vi "Main.vi"(11 "Module Admin":refnum<class "Delacor_lib_QMH_Module Admin.lvclass">) -> ()   [LabVIEW 2018, in "Log_class.lvlib"]
doc: "This template is based off of the Queued Message Handler design pattern and the Queued Message Handler project template that ships with LabVIEW.\n\nThe main difference is that the queue is private to this module and communication between modules is performed via Broadcast and Request events.\n\nRequest events are wrapped in public API methods and are handled in the Event Handling Loop (EHL) of this VI. Any module can register for Broadcast events sent by this module. The EHL generates messages based on user interface actions.\n\nThe Message Handling Loop (MHL) processes messages generated by the EHL, or by other messages. The messages are string values, so new messages can be added easily to the Message Cases case structure in the MHL. Each message cluster can also provide an optional value for Message Data, which is a variant that can be converted to whatever message-specific data is required.\n_____\nBased on DQMH Dev Tools: Project Template 7.1.1.1528."
uses:
  Log_class.lvlib
  <vilib>/Delacor/Delacor QMH/Libraries/Module Admin_class/Delacor_lib_QMH_Module Admin.lvclass
  Register_logs.ctl
  Module Data--cluster.ctl
  <vilib>/Delacor/Delacor QMH/Libraries/Message Queue_class/Delacor_lib_QMH_Message Queue.lvclass/Delacor_lib_QMH_Message Queue.ctl
  Stop Argument--cluster.ctl
  <vilib>/Delacor/Delacor QMH/Libraries/Module Admin_class/Delacor_lib_QMH_Module Admin.lvclass/Delacor_lib_QMH_Module Admin.ctl
  Log recording Argument--cluster.ctl
  Storage method changed Argument--cluster.ctl
  Request logs Argument--cluster.ctl
  Request logs (Reply Payload)--cluster.ctl
  Request save Argument--cluster.ctl
  <vilib>/Utility/miscctls.llb/LVPointTypeDef.ctl
  <vilib>/Delacor/Delacor QMH/Libraries/Message Queue_class/Delacor_lib_QMH_Enqueue Message (Single).vi
  <vilib>/Delacor/Delacor QMH/Libraries/Module Admin_class/Delacor_lib_QMH_Get External Launch.vi
  <vilib>/Delacor/Delacor QMH/Libraries/Message Queue_class/Delacor_lib_QMH_Message Queue.lvclass
panel:
  out "枚举":enum16{"自动存储", "触发式存储"}(ring)
  in  "组合框":T1
  out "error out":errorcluster
  out "Status":string
  in  "Simulate MHL Error":bool
  in  "Simulate EHL Error":bool
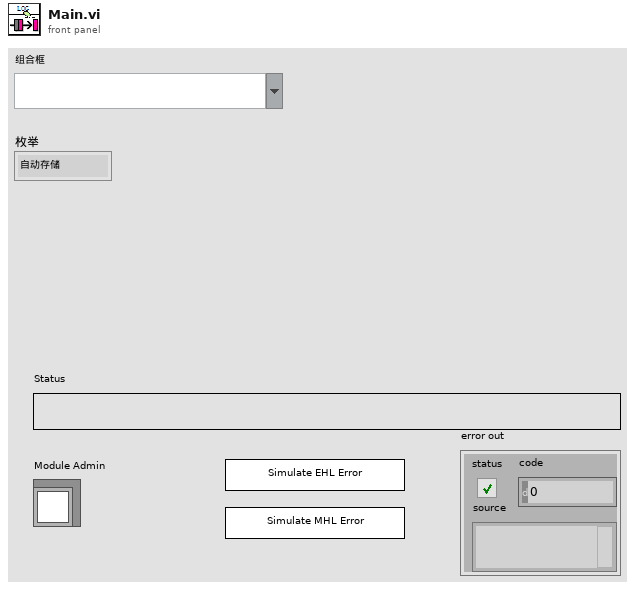
[diagram p1: front panel]
types:
  T1 = typedef "Log_class.lvlib/Register_logs.ctl" = string
  T2 = typedef "Log_class.lvlib/Request Events--cluster.ctl" = cluster{"Stop Module":refnum<user-event>, "Show Panel":refnum<user-event>, "Hide Panel":refnum<user-event>, "Get Module Execution Status":refnum<user-event>, "Show Diagram":refnum<user-event>, "记录日志":refnum<user-event>, "存储方式更改":refnum<user-event>, "请求日志":refnum<user-event>, "请求保存":refnum<user-event>}
  T3 = typedef "Log_class.lvlib/Module Data--cluster.ctl" = cluster{"Status":string, "创建的日志名":string[], "日志内容":string[], "存储方式":enum16{"自动存储", "触发式存储"}}
  T4 = enum32{"invalid lock state", "Not Locked", "Locked (No Password)", "Password-protected"}
  T5 = typedef "Log_class.lvlib/Stop Argument--cluster.ctl" = cluster{"Origin":string, "Exit via Stop Module Req?":bool, "Wait for Module to stop?":bool}
  T6 = typedef "Log_class.lvlib/Log recording Argument--cluster.ctl" = cluster{"日志选择":T1, "日志内容":string}
  T7 = typedef "Log_class.lvlib/Storage method changed Argument--cluster.ctl" = cluster{"枚举":enum16{"自动存储", "触发式存储"}}
  T8 = typedef "Log_class.lvlib/Request logs Argument--cluster.ctl" = cluster{"组合框":T1, "Wait Notifier":refnum<notifier>, "wait for reply":bool}
  T9 = typedef "Log_class.lvlib/Request save Argument--cluster.ctl" = cluster{"要保存的日志":T1}
  T10 = typedef "LVPointTypeDef.ctl" = cluster{"Horizontal":i16, "Vertical":i16}
  T11 = enum32{"Invalid", "Standard", "Closed", "Hidden", "Minimized", "Maximized"}
  T12 = typedef "Log_class.lvlib/Request logs (Reply Payload)--cluster.ctl" = cluster{"日志内容":string, "error":errorcluster}
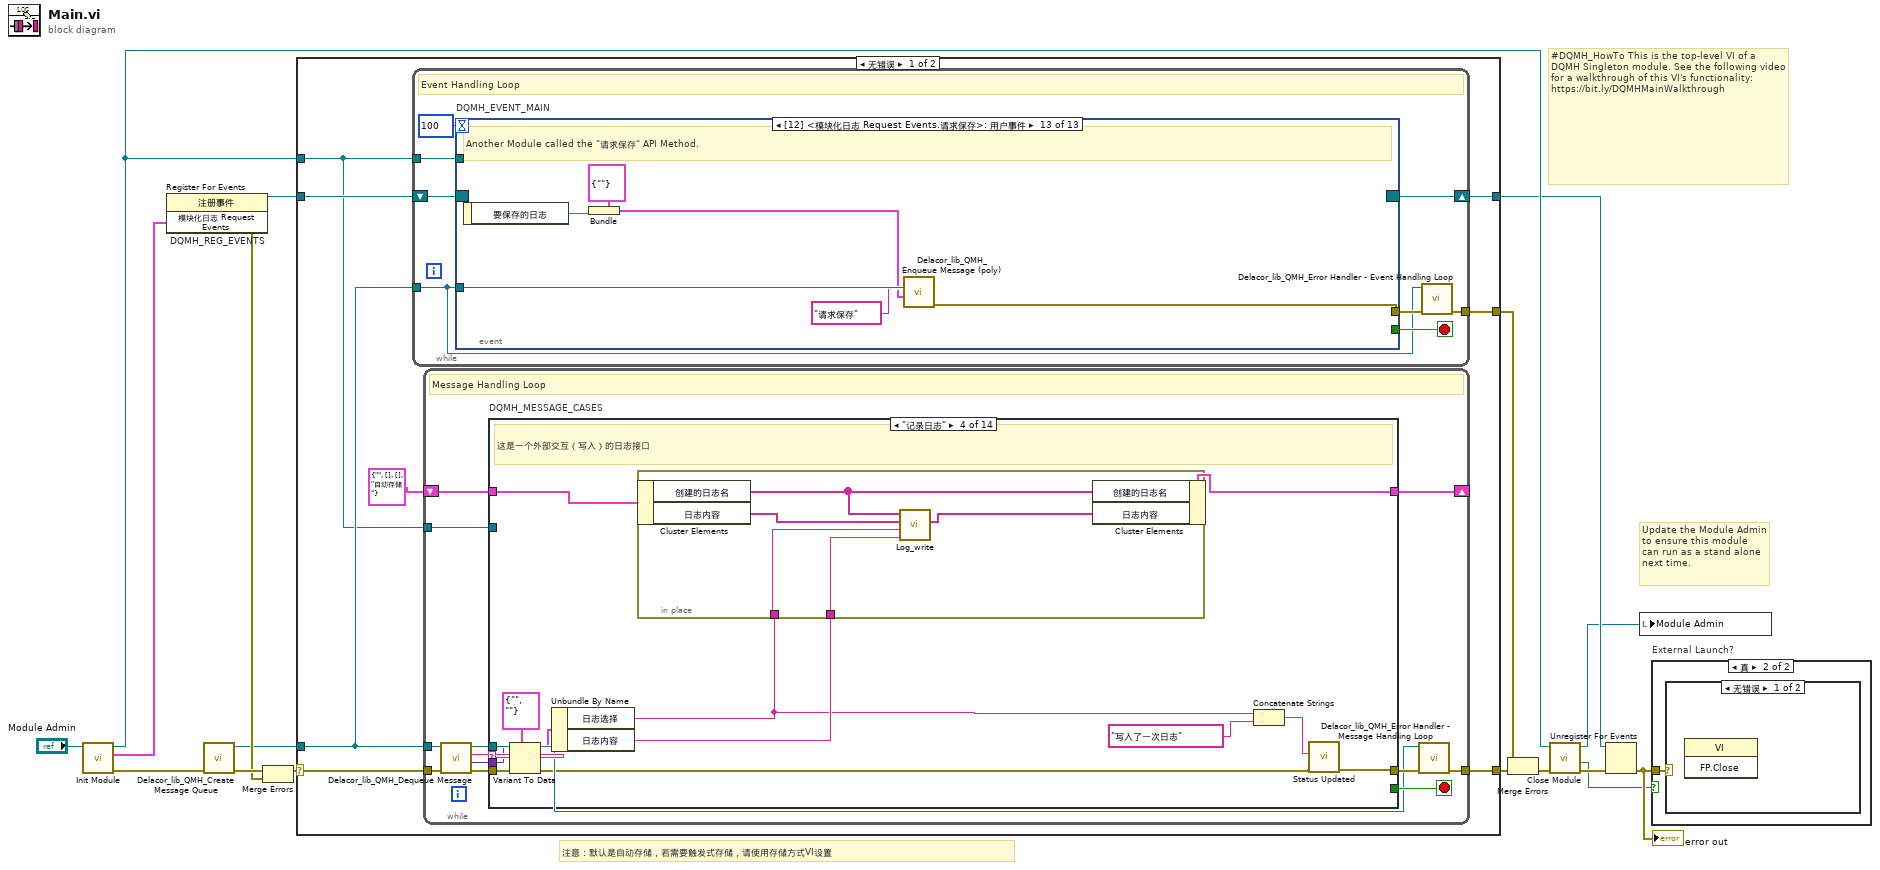
[diagram p0: block diagram]
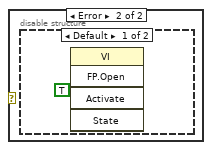
[diagram p3: hidden frame]
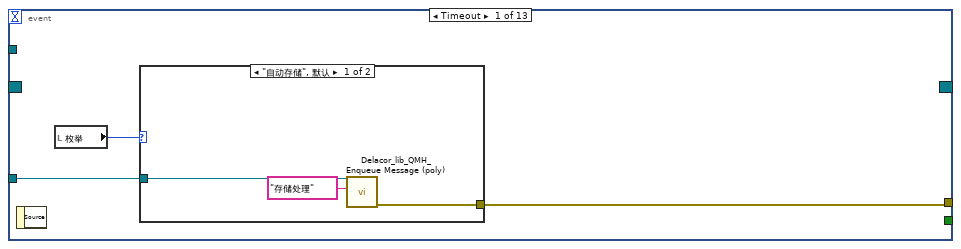
[diagram p5: hidden frame]
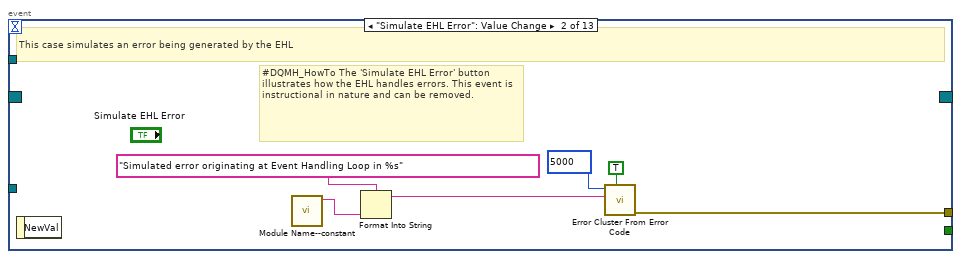
[diagram p7: hidden frame]
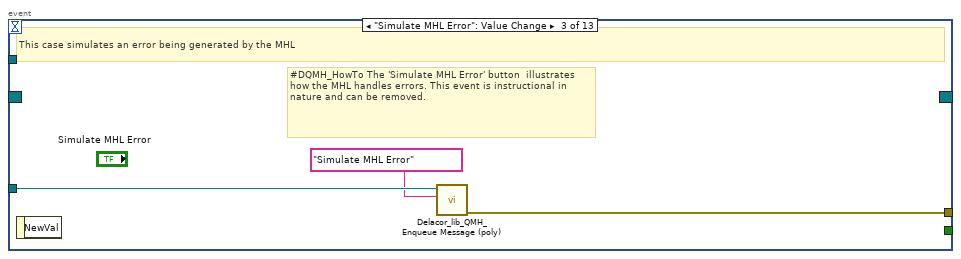
[diagram p8: hidden frame]
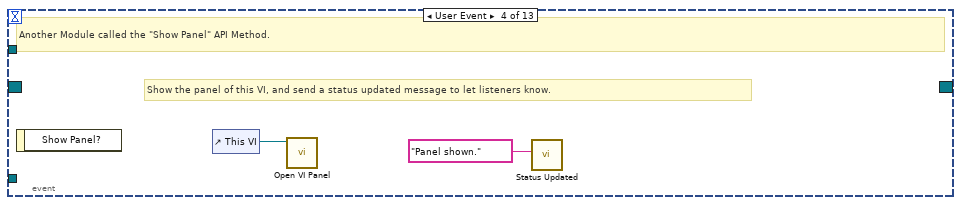
[diagram p9: hidden frame]
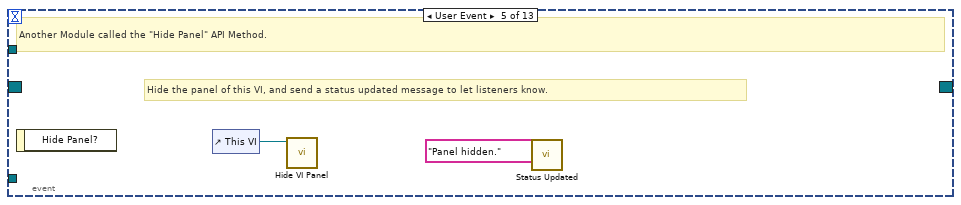
[diagram p10: hidden frame]
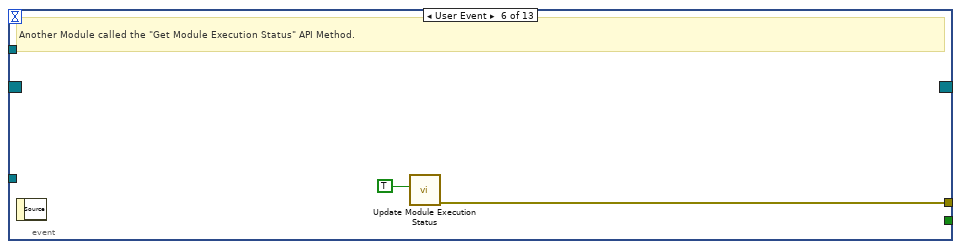
[diagram p11: hidden frame]
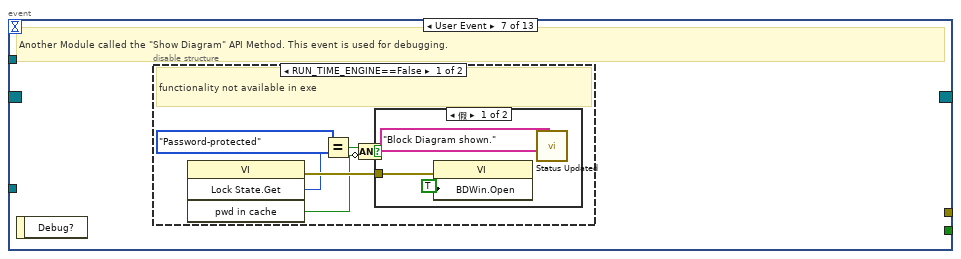
[diagram p12: hidden frame]
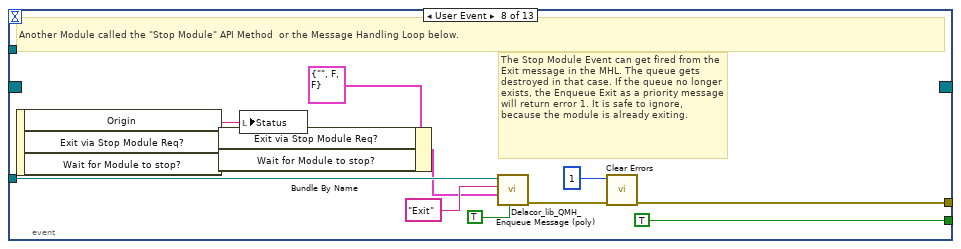
[diagram p15: hidden frame]
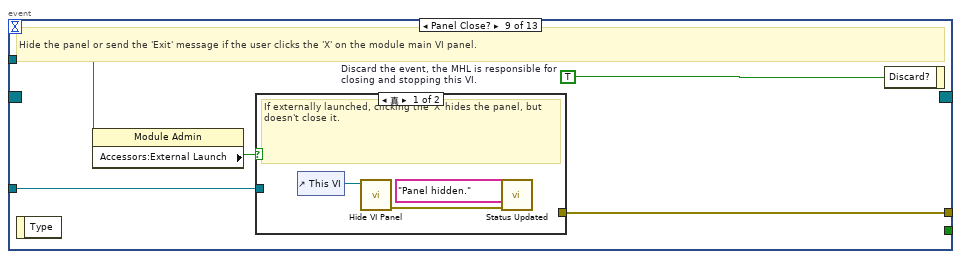
[diagram p16: hidden frame]
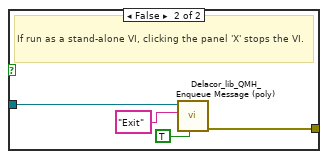
[diagram p17: hidden frame]
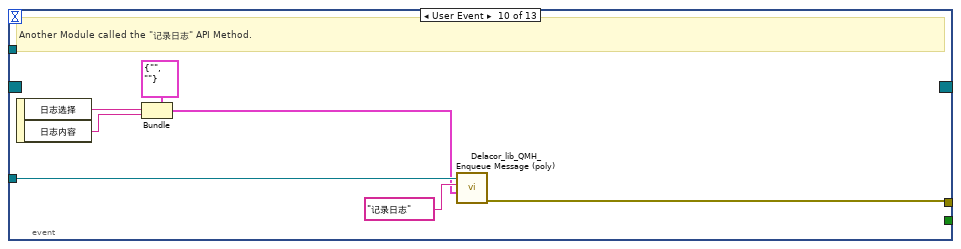
[diagram p18: hidden frame]
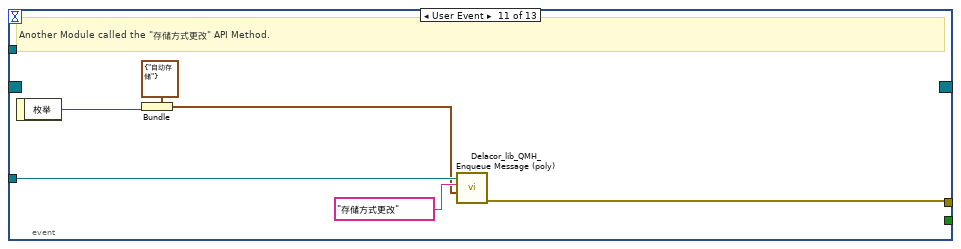
[diagram p19: hidden frame]
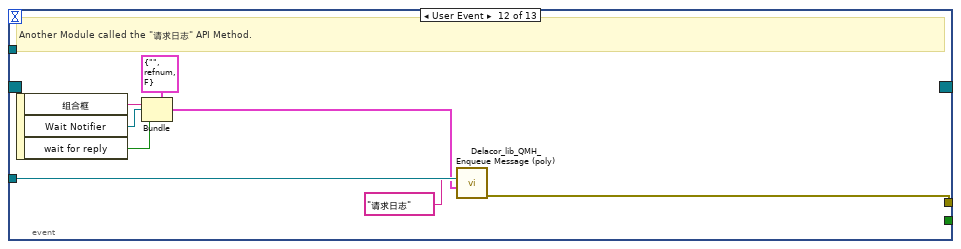
[diagram p20: hidden frame]
diagram:
  # "注意：默认是自动存储，若需要触发式存储，请使用存储方式VI设置"
  # "#DQMH_HowTo This is the top-level VI of a DQMH Singleton module. See the following video for a walkthrough of this VI's functionality: https://bit.ly/DQMHMainWalkthrough"
  # "Update the Module Admin to ensure this module can run as a stand alone next time."
  n1 = call "Init Module.vi"("Singleton Module Admin in"="Module Admin") -> ("error out"=w16:errorcluster, "模块化日志 Request Events"=w5:T2, "Singleton Module Admin out"=w8:refnum<class "Delacor_lib_QMH_Module Admin.lvclass">)  [unwired: 8 in]
  n2 = register-events "DQMH_REG_EVENTS"(w5) -> (reference out=w6:refnum<event-registration>, error out=w9:errorcluster)  [unwired: 2 in]
  n3 = call <vilib>:"Delacor_lib_QMH_Create Message Queue.vi"("error in"=w16) -> ("error out"=w11:errorcluster, "Message Queue"=w4:refnum<class "Delacor_lib_QMH_Message Queue.lvclass">)  [unwired: 9 in]
  n4 = Merge Errors(w11, w9) -> (w10:errorcluster)
  n5 = case shown="无错误" w10 {
    selector: w10 -> [w23 w297]
    tunnel: [w25 w296] -> w17
    tunnel: [w22 w295] -> w7
    tunnel: w6 -> [w20 w295]
    tunnel: w4 -> [w19 w290]
    tunnel: [w24 _] -> w14
    tunnel: w8 -> [w18 w291]
    frame No Error {
      n6 = while {
        tunnel: w19 -> [w27]
        shift-right: [w30] -> w22
        shift-left: w20 -> [w31]
        tunnel: [w32] -> w24
        tunnel: w18 -> [w28]
        stop <- w29 stop-if-true
        # "Event Handling Loop"
        n7 = event "DQMH_EVENT_MAIN" shown="[12] <模块化日志 Request Events.请求保存>: 用户事件" {
          selector: w31 -> [_ _ _ _ _ _ _ _ _ _ _ _ _]
          dyn-events: [_ _ _ _ _ _ _ _ _ _ _ _ _] -> w30
          timeout: 100 -> [_ _ _ _ _ _ _ _ _ _ _ _ _]
          tunnel: [_ _ _ _ _ _ _ TRUE ("Discard?") _ _ _ _ _] -> w29
          tunnel: w27 -> [w35 _ w47 _ _ _ _ w71 w78 w94 w100 w108 w114]
          tunnel: [w34 w45 w48 _ _ w54 _ w74 w80 w88 w95 w101 w109] -> w33
          tunnel: w28 -> [_ _ _ _ _ _ _ _ w77 _ _ _ _]
          event Timeout {
            n8 = event-data() -> ()  [unwired: 1 in, 1 out]
            n9 = local read "枚举"() -> (w36:enum16{"自动存储", "触发式存储"})
            n10 = case "条件结构" shown="\"自动存储\", 默认" w36 {
              tunnel: w35 -> [w39 _]
              tunnel: [w38 _] -> w34
              frame "自动存储", Default {
                n11 = call-poly <vilib>:"Delacor_lib_QMH_Enqueue Message (poly).vi"("Message"="存储处理", "Message Queue in"=w39) -> ("error out"=w38:errorcluster)  [unwired: 8 in, 1 out]
              }
              frame "触发式存储" {
              }
            }
          }
          event "Simulate EHL Error": Value Change {
            # "#DQMH_HowTo The 'Simulate EHL Error' button  illustrates how the EHL handles errors. This event is instructional in nature and can be removed."
            # "This case simulates an error being generated by the EHL"
            n12 = event-data() -> ()  [unwired: 1 in, 1 out]
            n13 = call "Module Name--constant.vi"() -> ("Module Name"=w42:string)  [unwired: 11 in]
            n14 = Format Into String(format string="Simulated error originating at Event Handling Loop in %s", w42) -> (resulting string=w43:string)  [unwired: 2 in, 1 out]
            n15 = call <vilib>:"Error Cluster From Error Code.vi"("show call chain? (False)"=TRUE, "error message (\"\")"=w43, "error code (0)"=5000) -> ("error out"=w45:errorcluster)  [unwired: 6 in]
          }
          event "Simulate MHL Error": Value Change {
            # "#DQMH_HowTo The 'Simulate MHL Error' button  illustrates how the MHL handles errors. This event is instructional in nature and can be removed."
            # "This case simulates an error being generated by the MHL"
            n16 = event-data() -> ()  [unwired: 1 in, 1 out]
            n17 = call-poly <vilib>:"Delacor_lib_QMH_Enqueue Message (poly).vi"("Message"="Simulate MHL Error", "Message Queue in"=w47) -> ("error out"=w48:errorcluster)  [unwired: 8 in, 1 out]
          }
          event User Event {
            # "Show the panel of this VI, and send a status updated message to let listeners know."
            # "Another Module called the \"Show Panel\" API Method."
            n18 = event-data() -> ()  [unwired: 1 in, 1 out]
            n19 = control-ref of="This VI"() -> (w50:refnum<vi>)
            n20 = call "Open VI Panel.vi"("VI"=w50) -> ()  [unwired: 10 in, 1 out]
            n21 = call "Status Updated.vi"("Status"="Panel shown." ("format string")) -> ()  [unwired: 10 in, 1 out]
          }
          event User Event {
            # "Hide the panel of this VI, and send a status updated message to let listeners know."
            # "Another Module called the \"Hide Panel\" API Method."
            n22 = event-data() -> ()  [unwired: 1 in, 1 out]
            n23 = control-ref of="This VI"() -> (w52:refnum<vi>)
            n24 = call "Hide VI Panel.vi"("VI"=w52) -> ()  [unwired: 10 in, 1 out]
            n25 = call "Status Updated.vi"("Status"="Panel hidden." ("format string")) -> ()  [unwired: 10 in, 1 out]
          }
          event User Event {
            # "Another Module called the \"Get Module Execution Status\" API Method."
            n26 = event-data() -> ()  [unwired: 1 in, 1 out]
            n27 = call "Update Module Execution Status.vi"("Running?"=TRUE) -> ("error out"=w54:errorcluster)  [unwired: 10 in]
          }
          event User Event {
            # "Another Module called the \"Show Diagram\" API Method. This event is used for debugging."
            n28 = event-data() -> ()  [unwired: 1 in, 1 out]
            n29 = disable-structure shown="RUN_TIME_ENGINE==False" {
              frame condition #0 (active) {
                # "functionality not available in exe"
                n30 = invoke on="Invoke Node" class="VI" method="Lock State.Get"() -> (error out=w60:errorcluster, "Get Lock State"=w59:T4, "pwd in cache"=w56:bool)  [unwired: 4 in, 1 out]
                n31 = Equal?(x=T4."Password-protected", y=w59) -> (x = y?=w57:bool)
                n32 = Compound Arithmetic op=AND(w57, invert w56) -> (w55:bool)
                n33 = case shown="假" w55 {
                  tunnel: w60 -> [w63 _]
                  frame False {
                    n34 = property on="Property Node" class="VI"(error in=w63, "BDWin.Open"=TRUE ("Block Diagram Window:Open")) -> ()  [unwired: 1 in, 2 out]
                    n35 = call "Status Updated.vi"("Status"="Block Diagram shown." ("format string")) -> ()  [unwired: 10 in, 1 out]
                  }
                  frame True {
                    # "Password-protected VI, and the password is not in the cache. Do not show the diagram."
                  }
                }
              }
              frame condition #1 {
              }
            }
          }
          event User Event {
            # "The Stop Module Event can get fired from the Exit message in the MHL. The queue gets destroyed in that case. If the queue no longer exists, the Enqueue Exit as a priority message will return error 1. It is safe to ignore, because the module is already exiting."
            # "Another Module called the \"Stop Module\" API Method  or the Message Handling Loop below."
            n36 = event-data() -> ("Origin"=w70:string, "Exit via Stop Module Req?"=w66:bool, "Wait for Module to stop?"=w65:bool)  [unwired: 1 in]
            n37 = Bundle By Name(cluster=T5 {"Origin"="", "Exit via Stop Module Req?"=FALSE, "Wait for Module to stop?"=FALSE} ("Stop Argument"), "Exit via Stop Module Req?"=w66, "Wait for Module to stop?"=w65) -> (w64:T5)
            n38 = local write "Status"(w70) -> ()
            n39 = call-poly <vilib>:"Delacor_lib_QMH_Enqueue Message (poly).vi"("Priority Message? (F)"=TRUE, "Message Data"=w64, "Message"="Exit", "Message Queue in"=w71) -> ("error out"=w75:errorcluster)  [unwired: 6 in, 1 out]
            n40 = call <vilib>:"Clear Errors.vi"("error in (no error)"=w75, "specific error code to clear (0: all)"=1) -> ("error out"=w74:errorcluster)  [unwired: 4 in, 1 out]
          }
          event Panel Close? {
            w79 = TRUE  # Discard the event, the MHL is responsible for closing and stopping this VI.
            # "Hide the panel or send the 'Exit' message if the user clicks the 'X' on the module main VI panel."
            n41 = event-data() -> ()  [unwired: 1 in, 1 out]
            n42 = property on="Property Node" class="Module Admin"(reference=w77) -> ("Accessors:External Launch"=w76:bool)  [unwired: 1 in, 2 out]
            n43 = case shown="真" w76 {
              tunnel: w78 -> [_ w86]
              tunnel: [_ w87] -> w80
              frame True {
                # "If externally launched, clicking the 'X' hides the panel, but doesn't close it."
                n44 = control-ref of="This VI"() -> (w83:refnum<vi>)
                n45 = call "Hide VI Panel.vi"("VI"=w83) -> ("error out"=w81:errorcluster)  [unwired: 10 in]
                n46 = call "Status Updated.vi"("error in"=w81, "Status"="Panel hidden." ("format string")) -> ()  [unwired: 9 in, 1 out]
              }
              frame False {
                # "If run as a stand-alone VI, clicking the panel 'X' stops the VI."
                n47 = call-poly <vilib>:"Delacor_lib_QMH_Enqueue Message (poly).vi"("Priority Message? (F)"=TRUE, "Message"="Exit", "Message Queue in"=w86) -> ("error out"=w87:errorcluster)  [unwired: 7 in, 1 out]
              }
            }
            n48 = event-data ("Event Filter Node")("Discard?"=w79) -> ()  [unwired: 1 in, 1 out]
          }
          event User Event {
            # "Another Module called the \"记录日志\" API Method."
            n49 = event-data() -> ("日志选择"=w90:T1, "日志内容"=w89:string)  [unwired: 1 in]
            n50 = Bundle(cluster=T6 {"日志选择"="", "日志内容"=""} ("记录日志 Argument"), "日志选择"=w90, "日志内容"=w89) -> (w91:T6)
            n51 = call-poly <vilib>:"Delacor_lib_QMH_Enqueue Message (poly).vi"("Message Data"=w91, "Message"="记录日志", "Message Queue in"=w94) -> ("error out"=w88:errorcluster)  [unwired: 7 in, 1 out]
          }
          event User Event {
            # "Another Module called the \"存储方式更改\" API Method."
            n52 = event-data() -> ("枚举"=w96:enum16{"自动存储", "触发式存储"})  [unwired: 1 in]
            n53 = Bundle(cluster=T7 {"枚举"=enum."自动存储"} ("存储方式更改 Argument"), "枚举"=w96) -> (w97:T7)
            n54 = call-poly <vilib>:"Delacor_lib_QMH_Enqueue Message (poly).vi"("Message Data"=w97, "Message"="存储方式更改", "Message Queue in"=w100) -> ("error out"=w95:errorcluster)  [unwired: 7 in, 1 out]
          }
          event User Event {
            # "Another Module called the \"请求日志\" API Method."
            n55 = event-data() -> ("组合框"=w104:T1, "Wait Notifier"=w103:refnum<notifier>, "wait for reply"=w102:bool)  [unwired: 1 in]
            n56 = Bundle(cluster=T8 {"组合框"="", "Wait Notifier"=refnum, "wait for reply"=FALSE} ("请求日志 Argument"), "组合框"=w104, "Wait Notifier"=w103, "wait for reply"=w102) -> (w105:T8)
            n57 = call-poly <vilib>:"Delacor_lib_QMH_Enqueue Message (poly).vi"("Message Data"=w105, "Message"="请求日志", "Message Queue in"=w108) -> ("error out"=w101:errorcluster)  [unwired: 7 in, 1 out]
          }
          event User Event {
            # "Another Module called the \"请求保存\" API Method."
            n58 = event-data() -> ("要保存的日志"=w110:T1)  [unwired: 1 in]
            n59 = Bundle(cluster=T9 {"要保存的日志"=""} ("请求保存 Argument"), "要保存的日志"=w110) -> (w111:T9)
            n60 = call-poly <vilib>:"Delacor_lib_QMH_Enqueue Message (poly).vi"("Message Data"=w111, "Message"="请求保存", "Message Queue in"=w114) -> ("error out"=w109:errorcluster)  [unwired: 7 in, 1 out]
          }
        }
        n61 = call-dynamic "Delacor_lib_QMH_Error Handler - Event Handling Loop.vi"("error in"=w33, "Message Queue in"=w27) -> ("dup error in"=w32:errorcluster)  [unwired: 8 in, 1 out]
      }
      n62 = while {
        tunnel: w19 -> [w115]
        shift-right: [w123] -> _
        shift-left: T3 {"Status"="", "创建的日志名"=[], "日志内容"=[], "存储方式"=enum."自动存储"} ("Data Cluster") -> [w124]
        tunnel: w23 -> [w126]
        tunnel: [w118] -> w25
        tunnel: w18 -> [w119]
        stop <- w122 stop-if-true
        # "Message Handling Loop"
        n63 = call-dynamic "Delacor_lib_QMH_Dequeue Message.vi"("error in"=w126, "Message Queue in"=w115) -> ("error out"=w125:errorcluster, "Message Data"=w120:variant, "Message"=w121:string, "Message Queue out"=w116:refnum<class "Delacor_lib_QMH_Message Queue.lvclass">)  [unwired: 6 in]
        n64 = case "DQMH_MESSAGE_CASES" shown="\"记录日志\"" w121 {
          selector: w121 -> [_ _ _ _ _ _ _ _ _ _ _ _ _ w285]
          tunnel: w116 -> [w128 _ _ _ _ _ _ _ _ _ _ w247 w271 _]
          tunnel: w125 -> [w147 w155 w159 w171 w184 w200 w212 w225 w229 w234 w243 w254 w277 w288]
          tunnel: [w146 w154 w159 w163 w182 w192 w207 w224 w228 w234 w242 w250 w272 w289] -> w117
          tunnel: w124 -> [w137 w157 w158 w167 w183 w191 w206 w223 w227 w233 w240 w249 w263 w286]
          tunnel: [w136 w151 w158 w166 w178 w191 w203 w223 w226 w233 w240 w249 w263 w286] -> w123
          tunnel: [_ _ _ _ _ _ _ _ _ _ _ _ w270 _] -> w122
          tunnel: w120 -> [_ _ _ w170 w181 w199 w210 _ _ _ _ w248 w269 _]
          tunnel: w119 -> [w138 _ _ _ _ _ _ _ _ _ _ w246 w264 _]
          frame "Initialize" {
            w132 = "Initial Message" ("Initial Message")
            # "Initialize - Any operation that needs to be done before the module can receive messages. Synchronize Caller Events.vi will inform Start Module.vi that the module has launched and is ready to receive messages. Module Did Init.vi will broadcast that the module initialized."
            n65 = call "Synchronize Caller Events.vi"("error in"=w147, "Singleton Module Admin in"=w138) -> ("error out"=w130:errorcluster, "Singleton Module Admin out"=w133:refnum<class "Delacor_lib_QMH_Module Admin.lvclass">)  [unwired: 8 in]
            n66 = property on="Property Node" class="Module Admin"(reference=w133) -> ("Accessors:External Launch"=w142:bool)  [unwired: 1 in, 2 out]
            n67 = Select(t=T11."Hidden" ("State"), s=w142, f=T11."Standard" ("State")) -> (s? t:f=w139:T11)
            n68 = call "Module Name--constant.vi"() -> ("Module Name"=w145:string)  [unwired: 11 in]
            n69 = property on="Property Node" class="VI"("Front Panel.Title"=w145) -> (reference out=w144:refnum<vi>, error out=w149:errorcluster)  [unwired: 2 in]
            n70 = invoke on="Invoke Node" class="VI" method="FP.Open"(reference=w144, error in=w149, "State"=w139) -> (reference out=w143:refnum<vi>, error out=w148:errorcluster)  [unwired: 2 in, 3 out]
            n71 = Bundle By Name(cluster=w137, "Status"=w132) -> (w136:T3)
            n72 = invoke on="Invoke Node" class="VI" method="FP.Center"(reference=w143, error in=w148) -> ()  [unwired: 1 in, 3 out]
            n73 = call-poly <vilib>:"Delacor_lib_QMH_Enqueue Message (poly).vi"("error in"=w130, "Message"="Init1", "Message Queue in"=w128) -> ("error out"=w129:errorcluster)  [unwired: 7 in, 1 out]
            n74 = property on="Pane" class="Pane"("Origin"=T10 {"Horizontal"=0, "Vertical"=0}) -> ()  [unwired: 2 in, 2 out]
            n75 = call "Module Name--constant.vi"() -> ("Module Name"=w134:string)  [unwired: 11 in]
            n76 = call "Module Did Init.vi"("error in"=w129, "Initialized?"=TRUE, "Origin"=w134) -> ("error out"=w146:errorcluster)  [unwired: 8 in]
            "Status" <- w132
          }
          frame "Init1" {
            n77 = property on="组合框" class="CmbBox (严格)"() -> ("Strings[]"=w153:string[])  [unwired: 2 in, 2 out]
            n78 = call "Init_log_array.vi"("要创建的日志名字"=w153) -> ("数组"=w152:string[])  [unwired: 10 in]
            n79 = Bundle By Name(cluster=w157, "创建的日志名"=w153, "日志内容"=w152) -> (w151:T3)
            n80 = Unbundle By Name(w151) -> ("存储方式"=w150:enum16{"自动存储", "触发式存储"})
            n81 = local write "枚举"(w150) -> ()
            n82 = call "Status Updated.vi"("error in"=w155, "Status"="注册成功" ("format string")) -> ("error out"=w154:errorcluster)  [unwired: 9 in]
          }
          frame "---Module Specific---" {
            # "Separator -- The following cases handle messages specific to this Module."
          }
          frame "记录日志" {
            # "这是一个外部交互（写入）的日志接口"
            n83 = Variant To Data(error in=w171, type=T6 {"日志选择"="", "日志内容"=""} ("记录日志 Argument"), Variant=w170) -> (data=w168:T6, error out=w164:errorcluster)
            n84 = Unbundle By Name(w168) -> ("日志选择"=w162:T1, "日志内容"=w165:string)
            n85 = in-place {
              in-place-border: w162 -> [w174]
              in-place-border: w165 -> [w173]
              n86 = in-place-cluster #1(w167) -> ("创建的日志名"=w176:string[], "日志内容"=w175:string[])
              n87 = call "Log_write.vi"("日志内容in 2"=w173, "日志选择"=w174, "日志内容in"=w175, "创建的日志"=w176) -> ("日志内容out"=w172:string[])  [unwired: 7 in]
              n88 = in-place-cluster #1("创建的日志名"=w176, "日志内容"=w172) -> (w166:T3)
            }
            n89 = Concatenate Strings(w162, "写入了一次日志" ("format string")) -> (w160:string)
            n90 = call "Status Updated.vi"("error in"=w164, "Status"=w160) -> ("error out"=w163:errorcluster)  [unwired: 9 in]
          }
          frame "存储方式更改" {
            # "#DQMH_CodeNeeded\n1. Configure this Message Case for handling the \"存储方式更改\" message.\n2. Delete or edit this label when done."
            # "存储方式更改"
            n91 = Variant To Data(error in=w184, type=T7 {"枚举"=enum."自动存储"} ("存储方式更改 Argument"), Variant=w181) -> (data=w179:T7, error out=w182:errorcluster)
            n92 = Unbundle By Name(w179) -> ("枚举"=w177:enum16{"自动存储", "触发式存储"})
            "枚举" <- w177
            n93 = Bundle By Name(cluster=w183, "存储方式"=w177) -> (w178:T3)
          }
          frame "请求日志" {
            # "#DQMH_CodeNeeded\n1. Configure this Message Case for handling the \"请求日志\" message.\n2. Wire any error that occurs to the \"error\" terminal.\n3. Delete or edit this label when done."
            # "获取当前的日志内容"
            n94 = Variant To Data(error in=w200, type=T8 {"组合框"="", "Wait Notifier"=refnum, "wait for reply"=FALSE} ("请求日志 Argument"), Variant=w199) -> (data=w197:T8, error out=w185:errorcluster)
            n95 = Unbundle By Name(w197) -> ("组合框"=w189:T1, "Wait Notifier"=w196:refnum<notifier>, "wait for reply"=w195:bool)
            n96 = Unbundle By Name(w191) -> ("创建的日志名"=w190:string[], "日志内容"=w188:string[])
            n97 = Search 1D Array(1D array=w190, element=w189) -> (index of element=w187:i32)  [unwired: 1 in]
            n98 = Index Array(array=w188, index=w187) -> (element=w186:string)
            n99 = Bundle By Name(cluster=T12 {"日志内容"="", "error"={"status"=FALSE, "code"=0, "source"=""}} ("请求日志 (Reply Payload)"), "日志内容"=w186, "error"=w185) -> (w194:T12)
            n100 = Merge Errors(w185) -> (w192:errorcluster)
            n101 = case "DQMH_FIRE_NOTIFIER" shown="真" w195 {
              tunnel: w196 -> [_ w202]
              tunnel: w194 -> [_ w201]
              frame False {
              }
              frame True {
                n102 = Send Notification(notification=w201, notifier=w202) -> ()  [unwired: 1 in, 2 out]
              }
            }
          }
          frame "请求保存" {
            # "发送一个请求去保存日志"
            n103 = Variant To Data(error in=w212, type=T9 {"要保存的日志"=""} ("请求保存 Argument"), Variant=w210) -> (data=w208:T9, error out=w211:errorcluster)
            n104 = Unbundle By Name(w208) -> ("要保存的日志"=w205:T1)
            n105 = in-place {
              in-place-border: w205 -> [w219]
              in-place-border: [w220] -> w204
              n106 = in-place-cluster #2(w206) -> ("日志内容"=w216:string[], "创建的日志名"=w222:string[])
              n107 = Search 1D Array(1D array=w222, element=w219) -> (index of element=w215:i32)  [unwired: 1 in]
              n108 = Build Array(w219) -> (w218:T1[])
              n109 = Index Array(array=w216, index=w215) -> (element=w221:string)
              n110 = call "Init_log_array.vi"("要创建的日志名字"=w218) -> ("数组"=w217:string[])  [unwired: 10 in]
              n111 = Index Array(array=w217) -> (element=w214:string)  [unwired: 1 in]
              n112 = call "Local_write.vi"("内容"=w221, "名字"=w219) -> ("错误输出"=w220:errorcluster)  [unwired: 9 in]
              n113 = Replace Array Subset(array=w216, new element=w214, index=w215) -> (w213:string[])
              n114 = in-place-cluster #2("日志内容"=w213, "创建的日志名"=w222) -> (w203:T3)
            }
            n115 = Merge Errors(w204, w211) -> (w207:errorcluster)
          }
          frame "---Copy This Frame---" {
            # "Duplicate this frame when creating new messages.  Change this comment in the duplicated frame to describe this message."
            n116 = Merge Errors(w225) -> (w224:errorcluster)
          }
          frame "存储处理" {
            # "Duplicate this frame when creating new messages.  Change this comment in the duplicated frame to describe this message."
            n117 = in-place {
              n118 = in-place-cluster #3(w227) -> ("创建的日志名"=w230:string[], "日志内容"=w232:string[])
              n119 = call "Judgment_based_storage.vi"("日志内容"=w232, "日志名"=w230) -> ("新日志数组"=w231:string[])  [unwired: 9 in]
              n120 = in-place-cluster #3("创建的日志名"=w230, "日志内容"=w231) -> (w226:T3)
            }
            n121 = Merge Errors(w229) -> (w228:errorcluster)
          }
          frame "---Exit and Error Handling---" {
            # "Separator - The following cases handle errors and exit messages."
          }
          frame "Simulate MHL Error" {
            # "#DQMH_HowTo The 'Simulate MHL Error' button  illustrates how the MHL handles errors. This event is instructional in nature and can be removed."
            # "Simulate an error occurring at the MHL"
            n122 = call "Module Name--constant.vi"() -> ("Module Name"=w236:string)  [unwired: 11 in]
            n123 = Format Into String(format string="Simulated error originating at Message Handling Loop in %s", w236) -> (resulting string=w237:string)  [unwired: 2 in, 1 out]
            n124 = call <vilib>:"Error Cluster From Error Code.vi"("show call chain? (False)"=TRUE, "error message (\"\")"=w237, "error code (0)"=5001) -> ("error out"=w241:errorcluster)  [unwired: 6 in]
            n125 = Merge Errors(w243, w241) -> (w242:errorcluster)
          }
          frame "Error" {
            # "#DQMH_CodeRecommended - If the module is running in standalone mode (External Launch = FALSE), this code will pop up an error dialog and call the 'Exit' message if an error occurs. Add more fine-grained error management here."
            # "Error - Check the error message data and respond accordingly. This message is sent by the \"Error Handler\" VIs at the end of each loop in this application."
            n126 = property on="Property Node" class="Module Admin"(reference=w246) -> ("Accessors:External Launch"=w245:bool)  [unwired: 1 in, 2 out]
            n127 = Variant To Data(error in=w254, type=errorcluster {"status"=FALSE, "code"=0, "source"=""} ("error constant"), Variant=w248) -> (data=w244:errorcluster, error out=w252:errorcluster)
            n128 = local write "error out"(w244) -> ()
            n129 = call "Error Reported.vi"("Error"=w244) -> ()  [unwired: 10 in, 1 out]
            n130 = case shown="假" w245 {
              tunnel: [w259 _] -> w251
              tunnel: w247 -> [w257 _]
              tunnel: w244 -> [w258 _]
              frame False {
                n131 = disable-structure shown="Default" {
                  disable-tunnel: w258 -> [w260 _]
                  frame condition #0 (active) {
                    # "If the module is running standalone, then pop up an error dialog and call the \"Exit\" message."
                    n132 = call <vilib>:"Simple Error Handler.vi"("error in (no error)"=w260) -> ()  [unwired: 4 in, 5 out]
                  }
                  frame condition #1 {
                    # "To prevent the Simple Error Handler VI from being loaded (e.g. when deploying to a Real-Time target), add the Conditional Disable Symbol \"DQMH_Disable_SEH\" to your project and set it to TRUE."
                  }
                }
                n133 = call-poly <vilib>:"Delacor_lib_QMH_Enqueue Message (poly).vi"("Priority Message? (F)"=TRUE, "Message"="Exit", "Message Queue in"=w257) -> ("error out"=w259:errorcluster)  [unwired: 7 in, 1 out]
              }
              frame True {
                # "If the module was launched externally, calling the Error Reported broadcast VI is the only action performed by the \"Error\" message. The module's caller can then process the error appropriately."
              }
            }
            n134 = Merge Errors(w252, w251) -> (w250:errorcluster)
          }
          frame "Exit" {
            w268 = 91  # 91: not all Exit messages will have an argument
            w270 = TRUE  # Stop the VI
            # "Release the message queue reference"
            # "Exit - Exit the application."
            n135 = Variant To Data(error in=w277, type=T5 {"Origin"="", "Exit via Stop Module Req?"=FALSE, "Wait for Module to stop?"=FALSE} ("Stop Argument"), Variant=w269) -> (data=w266:T5, error out=w274:errorcluster)
            n136 = call <vilib>:"Clear Errors.vi"("error in (no error)"=w274, "specific error code to clear (0: all)"=w268) -> ("error out"=w276:errorcluster)  [unwired: 4 in, 1 out]
            n137 = control-ref of="This VI"() -> (w265:refnum<vi>)
            n138 = call-dynamic "Delacor_lib_QMH_Release Message Queue.vi"("error in"=w276, "Message Queue"=w271) -> ("error out"=w275:errorcluster)  [unwired: 9 in]
            n139 = call "Handle Exit.vi"("Stop Argument"=w266, "Admin in"=w264, "VI reference"=w265) -> ("error out"=w273:errorcluster)  [unwired: 7 in, 1 out]
            n140 = Unbundle By Name(w263) -> ("创建的日志名"=w262:string[], "日志内容"=w261:string[])
            n141 = Merge Errors(w275, w273) -> (w272:errorcluster)
            n142 = call "Error Reported.vi"("Error"=w272) -> ()  [unwired: 10 in, 1 out]
            n143 = for {
              tunnel: w262 -> [w279] mode=indexing
              tunnel: w261 -> [w278] mode=indexing
              n144 = call "Local_write.vi"("内容"=w278, "名字"=w279) -> ()  [unwired: 9 in, 1 out]
            }
          }
          frame Default {
            # "'Default' case only runs if there is a message that isn't defined in any of the other cases.  Output a programming error."
            n145 = call "Module Name--constant.vi"() -> ("Module Name"=w284:string)  [unwired: 11 in]
            n146 = Format Into String(format string="The invalid message string \"%s\" was received in the Message Handling Loop for module \"%s\".", w285, w284) -> (resulting string=w280:string)  [unwired: 2 in, 1 out]
            n147 = call <vilib>:"Error Cluster From Error Code.vi"("show call chain? (False)"=TRUE, "error message (\"\")"=w280, "error code (0)"=1) -> ("error out"=w287:errorcluster)  [unwired: 6 in]
            n148 = Merge Errors(w288, w287) -> (w289:errorcluster)
          }
        }
        n149 = call-dynamic "Delacor_lib_QMH_Error Handler - Message Handling Loop.vi"("error in"=w117, "Message Queue in"=w116) -> ("dup error in"=w118:errorcluster)  [unwired: 8 in, 1 out]
      }
    }
    frame Error {
      # "Synchronize Caller Events.vi will inform Start Module.vi that the module has launched and will let the code calling Start Module.vi register for broadcasts and would permit the caller receive the broadcast that an error occurred at launch time."
      n150 = call-dynamic "Delacor_lib_QMH_Release Message Queue.vi"("error in"=w297, "Message Queue"=w290) -> ("error out"=w296:errorcluster)  [unwired: 9 in]
      n151 = call "Synchronize Caller Events.vi"("Singleton Module Admin in"=w291) -> ("error out"=w298:errorcluster)  [unwired: 9 in, 1 out]
      n152 = call "Module Name--constant.vi"() -> ("Module Name"=w294:string)  [unwired: 11 in]
      n153 = Format Into String(format string="An error occurred during initialization. %s is no longer running.", w294) -> (resulting string=w292:string)  [unwired: 2 in, 1 out]
      n154 = Merge Errors(w296, w298) -> (w299:errorcluster)
      n155 = call "Error Reported.vi"("Additional Information"=w292, "Error"=w299) -> ()  [unwired: 9 in, 1 out]
    }
  }
  n156 = Merge Errors(w14, w17) -> (w13:errorcluster)
  n157 = call "Close Module.vi"("error in"=w13, "Module Admin in"=w8) -> ("error out"=w15:errorcluster, "External Launch"=w1:bool, "Module Admin out"=w2:refnum<class "Delacor_lib_QMH_Module Admin.lvclass">)  [unwired: 7 in]
  n158 = Unregister For Events(event registration refnum=w7, error in=w15) -> (error out=w12:errorcluster)
  "error out" <- w12
  n159 = local write "Module Admin"(w2) -> ()
  n160 = case "External Launch?" shown="真" w1 {
    tunnel: w12 -> [_ w300]
    frame False {
    }
    frame True {
      n161 = case shown="无错误" w300 {
        frame No Error {
          n162 = invoke on="Invoke Node" class="VI" method="FP.Close"() -> ()  [unwired: 3 in, 3 out]
        }
        frame Error {
          n163 = disable-structure shown="Default" {
            frame condition #0 (active) {
              n164 = invoke class="VI" method="FP.Open"("Activate"=TRUE ("Activate?")) -> ()  [unwired: 4 in, 5 out]
            }
            frame condition #1 {
              # "Don't show panel on error if running inside a built EXE."
            }
          }
        }
      }
    }
  }
